vi "[ce] Eval y=f(a,x1,x2).vi"(6 "parameters":cluster{"name":string, "value":dbl}[](array[cluster]) {"value" format="%.2f"}, 7 "# points":u32=25, 8 "error in":errorcluster, 9 "formula info":T1={"formula"="", "variable 1"="x1", "variable 2"="x2"}, 10 "End":cluster{"x1":dbl, "x2":dbl}={"x1"=1.0, "x2"=1.0} {"x2" format="%.2f"; "x1" format="%.2f"}, 11 "Start":cluster{"x1":dbl, "x2":dbl} {"x2" format="%.2f"; "x1" format="%.2f"}) -> (0 "error out":errorcluster, 1 "Y Values":dbl[][](array[numeric]) format="%.2f", 2 "X2  Values":dbl[](array[numeric]) format="%.2f", 3 "X1 Values":dbl[](array[numeric]) format="%.2f", 4 "ticks":u32)   [LabVIEW 2021]
doc: "Calculates a 2D array of function values defined on a grid. In addition, the VI allows specifying additional parameters and evaluating them in formula.\n\n::: CalcExpress Toolkit :::\nCopyright (c) 2000-2026 Konstantin Shifershteyn. All rights reserved."
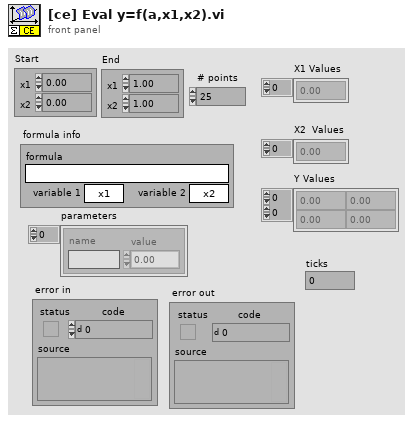
[diagram p1: front panel]
types:
  T1 = cluster{"formula":string, "variable 1":string, "variable 2":string}
  T2 = enum16{"create", "destroy", "set value", "get value"}
  T3 = typedef "VarMan Variable Context Handle.ctl" = i32
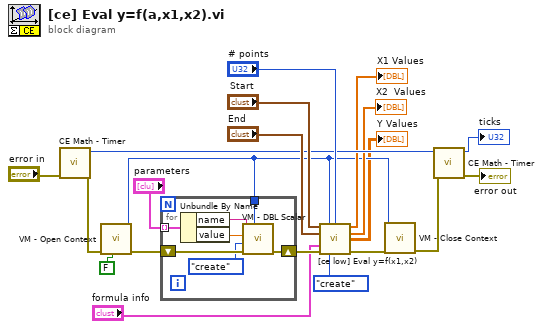
[diagram p0: block diagram]
diagram:
  n1 = call "CE Math - Timer.vi"("error in (no error)"="error in") -> ("error out"=w15:errorcluster, "ticks out"=w16:u32)  [unwired: 7 in]
  n2 = call "VM - Open Context.vi"("close loose contexts (F)"=FALSE ("close loose contexts (T)"), "error in"=w15) -> ("error out"=w10:errorcluster, "VC Handle out"=w3:T3)  [unwired: 7 in, 1 out]
  n3 = for {
    shift-right: [w24] -> w11
    shift-left: w10 -> [w25]
    tunnel: "parameters" -> [w22] mode=indexing
    tunnel: w3 -> [w21]
    n4 = Unbundle By Name(w22) -> ("name"=w26:string, "value"=w27:dbl)
    n5 = call "VM - DBL Scalar.vi"("VC Handle"=w21, "error in"=w25, "cmd"=T2."create", "value in"=w27, "name_spec"=w26) -> ("error out"=w24:errorcluster)  [unwired: 1 in, 5 out]
  }
  n6 = call "[ce low] Eval y=f(x1,x2).vi"("Start"="Start", "VC Handle"=w3, "number of points"="# points", "End"="End", "formula info"="formula info", "error in"=w11, "vm cmd"=T2."create") -> ("X1 Values"=→"X1 Values":dbl[], "X2  Values"=→"X2  Values":dbl[], "Y Values"=→"Y Values":dbl[][], "error out"=w20:errorcluster)  [unwired: 5 in]
  n7 = call "VM - Close Context.vi"("error in"=w20, "VC Handle"=w3) -> ("error out"=w13:errorcluster)  [unwired: 8 in, 1 out]
  n8 = call "CE Math - Timer.vi"("error in (no error)"=w13, "ticks in"=w16) -> ("error out"=→"error out":errorcluster, "ticks out"=→"ticks":u32)  [unwired: 6 in]
